vi "zadanie3_lab0.vi"() -> ()   [LabVIEW 2020]
uses:
  <vilib>/numeric/Random Number (Range) U64.vi
  <vilib>/numeric/sub_Random U32.vi
panel:
  out "output cluster":T1
  in  "input cluster 2":T1
  out "XY Graph":T2(graph)
  in  "liczba iteracji":dbl
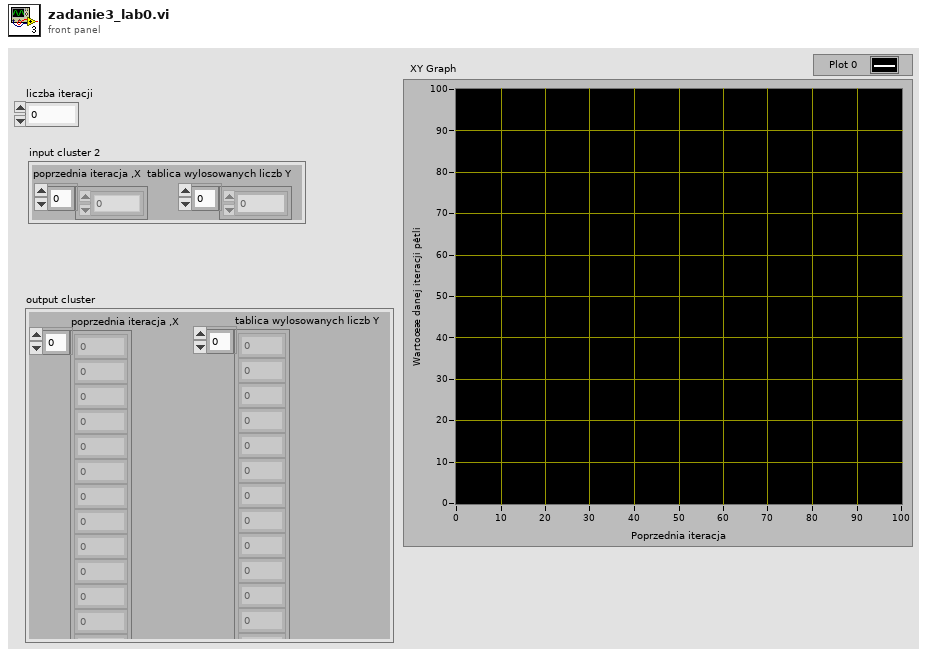
[diagram p1: front panel]
types:
  T1 = cluster{"tablica wylosowanych liczb Y":dbl[], "poprzednia iteracja ,X":dbl[]}
  T2 = cluster{"tablica wylosowanych liczb":dbl[], "iteracje":dbl[]}
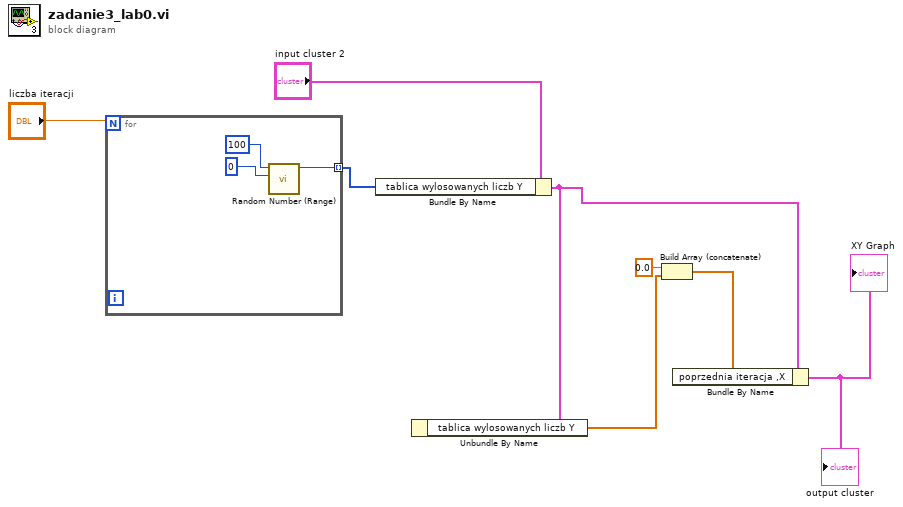
[diagram p0: block diagram]
diagram:
  n1 = for {
    N: "liczba iteracji" -> [_]
    tunnel: [w9] -> w6 mode=indexing
    n2 = call-poly <vilib>:"Random Number (Range).vi"("lower bound (0)"=u64 0, "upper bound (100)"=u64 100) -> ("number"=w9:u64)  [unwired: 9 in]
  }
  n3 = Bundle By Name(cluster="input cluster 2", "tablica wylosowanych liczb Y"=w6) -> (w4:T1)
  n4 = Unbundle By Name(w4) -> ("tablica wylosowanych liczb Y"=w2:dbl[])
  n5 = Build Array (concatenate)(0.0 ("element"), w2) -> (w1:dbl[])
  n6 = Bundle By Name(cluster=w4, "poprzednia iteracja ,X"=w1) -> (→"XY Graph" →"output cluster":T1)
